vi "SC Find Add-ons.vi"(8 "error in (no error)":errorcluster, 9 "entry VI":path) -> (0 "error out":errorcluster, 1 "add-on directories":string[](array[string]))   [LabVIEW 2023]
doc: "Loads the entry VI (and so its subVIs), then returns the add-on directories (.../LVAddons/<name>) of the VIs in memory that live in an LVAddons folder, except this deploy tool's own add-on."
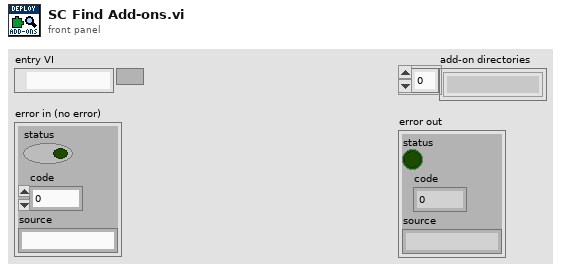
[diagram p1: front panel]
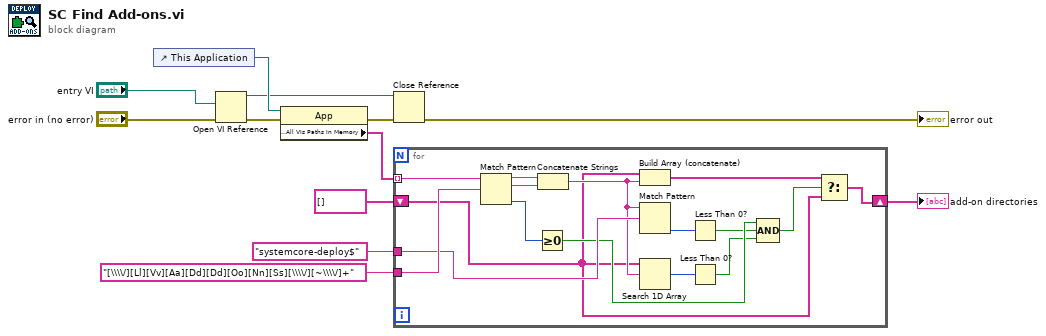
[diagram p0: block diagram]
diagram:
  n1 = control-ref of="This Application"() -> (w10:refnum<vi>)
  n2 = Open VI Reference(vi path="entry VI", error in (no error)="error in (no error)") -> (vi reference=w3:refnum<vi>, error out=w9:errorcluster)  [unwired: 4 in]
  n3 = property class="App"(reference=w10, error in=w9) -> (error out=w2:errorcluster, "Application:All VIs Paths In Memory"=w8:string[])  [unwired: 1 out]
  n4 = Close Reference(reference=w3, error in (no error)=w2) -> (error out=→"error out":errorcluster)
  n5 = for {
    tunnel: w8 -> [w28] mode=indexing
    tunnel: "[\\\\/][Ll][Vv][Aa][Dd][Dd][Oo][Nn][Ss][\\\\/][~\\\\/]+" -> [w27]
    tunnel: "systemcore-deploy$" -> [w23]
    shift-right: [w13] -> w5
    shift-left: string[] [] -> [w14]
    n6 = Match Pattern(string=w28, regular expression=w27) -> (before substring=w26:string, match substring=w25:string, offset past match=w24:i32)  [unwired: 1 in, 1 out]
    n7 = Greater Or Equal To 0?(x=w24) -> (x >= 0?=w20:bool)
    n8 = Concatenate Strings(w26, w25) -> (w17:string)
    n9 = Build Array (concatenate)(w14, w17) -> (w15:string[])
    n10 = Match Pattern(string=w17, regular expression=w23) -> (offset past match=w22:i32)  [unwired: 1 in, 3 out]
    n11 = Search 1D Array(1D array=w14, element=w17) -> (index of element=w21:i32)  [unwired: 1 in]
    n12 = Less Than 0?(x=w22) -> (x < 0?=w19:bool)
    n13 = Less Than 0?(x=w21) -> (x < 0?=w18:bool)
    n14 = Compound Arithmetic op=AND(w20, w19, w18) -> (w16:bool)
    n15 = Select(t=w15, s=w16, f=w14) -> (s? t:f=w13:string[])
  }
  "add-on directories" <- w5
